vi "Tell Child.vi"(4 "Priority":bool, 6 "UID":string, 7 "Actor in":refnum<class "Actor.lvclass">, 8 "Error in":errorcluster, 9 "Reply":bool, 10 "Msg":refnum<class "Msg.lvclass">) -> (0 "Error out":errorcluster, 5 "Actor out":refnum<class "Actor.lvclass">)   [LabVIEW 2020, in "jettl.lvlib"]
uses:
  jettl.lvlib
  Msg/Msg.lvclass
  Actor/Actor.lvclass
  Relation.ctl
  Base Teller/Base Teller/Base Teller.lvclass/Base Teller.ctl
  Base Teller/Init Teller.vi
  Default Implementation.vi
  Base Teller/Base Teller/Init Teller.vi
  Base Teller/Base Teller/Base Teller.lvclass
  C:/git/jettl/src/jettl/jettl/Teller/Teller.lvclass
  UID Not Found--error.vi
  Msg Input/Msg Input.lvclass
  Attributes/Attributes.lvclass
  Transport/Transport.lvclass
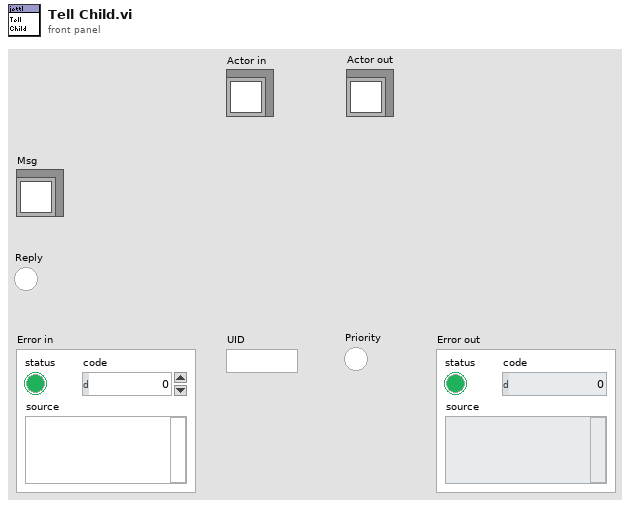
[diagram p1: front panel]
types:
  T1 = typedef "jettl.lvlib/Relation.ctl" = enum16{"Self", "Parent", "Child", "No Relation"}
  T2 = typedef "jettl.lvlib/Msgs.ctl" = set{refnum<class "Msg.lvclass">}
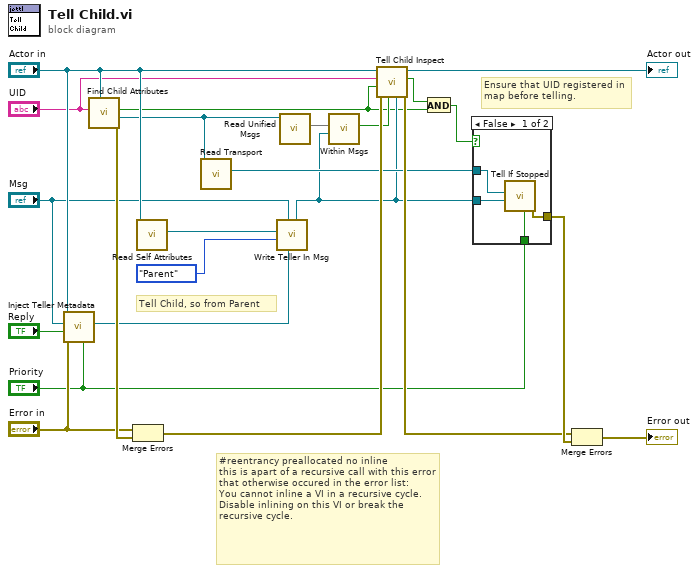
[diagram p0: block diagram]
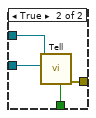
[diagram p2: hidden frame]
diagram:
  # "#reentrancy preallocated no inline\nthis is apart of a recursive call with this error that otherwise occured in the error list:\nYou cannot inline a VI in a recursive cycle. Disable inlining on this VI or break the recursive cycle."
  # "Ensure that UID registered in map before telling."
  # "Tell Child, so from Parent"
  n1 = call-dynamic "Inject Teller Metadata.vi"("Priority"="Priority", "Error in"="Error in", "Reply"="Reply", "Msg"="Msg", "Actor in"="Actor in") -> ("Teller Metadata"=w5:refnum<class "Teller Metadata.lvclass">)  [unwired: 6 in]
  n2 = call "Find Child Attributes.vi"("Actor in"="Actor in", "UID"="UID") -> ("Error out"=w7:errorcluster, "Child Attributes"=w14:refnum<class "Attributes.lvclass">, "Found"=w6:bool)  [unwired: 7 in]
  n3 = Merge Errors("Error in", w7) -> (w21:errorcluster)
  n4 = call-dynamic "Read Self Attributes.vi"("Actor in"="Actor in") -> ("Self Attributes"=w19:refnum<class "Attributes.lvclass">)  [unwired: 10 in]
  n5 = call-dynamic "Read Transport.vi"("Attributes in"=w14) -> ("Transport"=w13:refnum<class "Transport.lvclass">)  [unwired: 10 in]
  n6 = call "Write Teller In Msg.vi"("Teller Metadata"=w5, "Msg in"="Msg", "Relation"=Relation."Parent", "Attributes"=w19) -> ("Msg out"=w12:refnum<class "Msg.lvclass">)  [unwired: 7 in]
  n7 = call-dynamic "Read Unified Msgs.vi"("Attributes in"=w14) -> ("Unified Msgs"=w15:T2)  [unwired: 10 in]
  n8 = call "Within Msgs.vi"("Msg"=w12, "Msgs"=w15) -> ("Within Msgs"=w11:bool)  [unwired: 9 in]
  n9 = call-dynamic "Tell Child Inspect.vi"("Msg"=w12, "Within Unified Msgs"=w11, "Error in"=w21, "Found"=w6, "UID"="UID", "Actor in"="Actor in") -> ("Error out"=w20:errorcluster, "Proceed"=w9:bool, "Actor out"=→"Actor out":refnum<class "Actor.lvclass">)  [unwired: 3 in]
  n10 = And(x=w9, y=w6) -> (x .and. y?=w8:bool)
  n11 = case shown="False" w8 {
    tunnel: [w24 w31] -> w22
    tunnel: "Priority" -> [w25 w30]
    tunnel: w13 -> [w27 w29]
    tunnel: w12 -> [w26 w28]
    frame False {
      n12 = call "Tell If Stopped.vi"("Priority"=w25, "Msg"=w26, "Transport"=w27) -> ("Error out"=w24:errorcluster)  [unwired: 8 in]
    }
    frame True {
      n13 = call-dynamic "Tell.vi"("Priority"=w30, "Msg"=w28, "Transport in"=w29) -> ("Error out"=w31:errorcluster)  [unwired: 8 in]
    }
  }
  n14 = Merge Errors(w20, w22) -> (→"Error out":errorcluster)
